vi "Kappa.vi"() -> ()   [LabVIEW 2026]
doc: "Clamp x into the range [lo, hi]: returns hi when x is above hi, lo when x is below lo, and x otherwise. Two nested Case Structures, primitives only."
panel:
  out "clamped":dbl
  in  "hi":dbl=10.0
  in  "lo":dbl
  in  "x":dbl
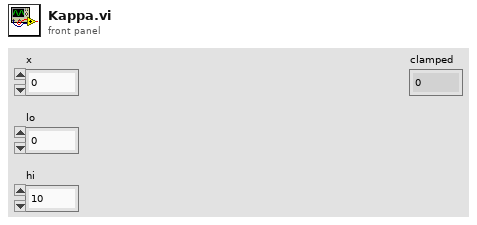
[diagram p1: front panel]
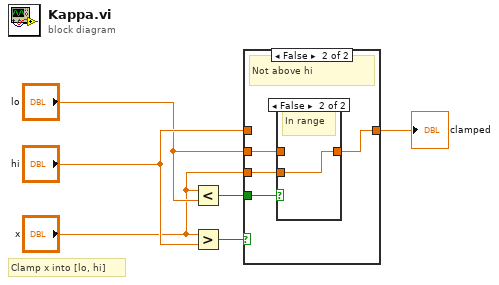
[diagram p0: block diagram]
diagram:
  # "Clamp x into [lo, hi]"
  n1 = Less?(x="x", y="lo") -> (x < y?=w3:bool)
  n2 = Greater?(x="x", y="hi") -> (0:w2:bool)
  n3 = case shown="False" w2 {
    tunnel: [w7 w8] -> w1
    tunnel: "hi" -> [w7 _]
    tunnel: "lo" -> [_ w11]
    tunnel: "x" -> [_ w10]
    tunnel: w3 -> [_ w9]
    frame True {
      # "Above hi"
    }
    frame False {
      # "Not above hi"
      n4 = case shown="False" w9 {
        tunnel: [w12 w13] -> w8
        tunnel: w11 -> [w12 _]
        tunnel: w10 -> [_ w13]
        frame True {
          # "Below lo"
        }
        frame False {
          # "In range"
        }
      }
    }
  }
  "clamped" <- w1
